vi "Set All Plot Visibility (WFGraph).vi"(8 "error in (no error)":errorcluster, 10 "All Visible?":bool, 11 "WFGraph in":refnum<vi>) -> (0 "error out":errorcluster)   [LabVIEW 2019, in "Instrument.Lockin.lvlib" / "Instrument UI.Lockin.lvclass"]
uses:
  Instrument UI.Lockin.lvclass
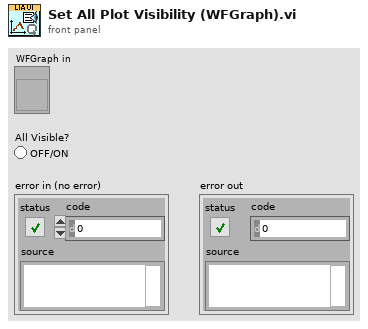
[diagram p1: front panel]
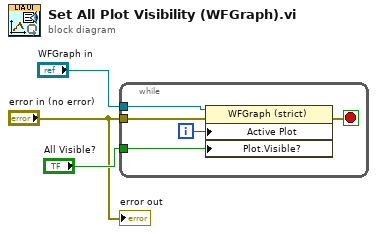
[diagram p0: block diagram]
diagram:
  n1 = while {
    tunnel: "WFGraph in" -> [w5]
    tunnel: "error in (no error)" -> [w6]
    tunnel: "All Visible?" -> [w7]
    i -> [w8]
    stop <- w4 stop-if-true
    n2 = property on="Property Node" class="WFGraph (strict)"(reference=w5, error in=w6, "Active Plot"=w8, "Plot.Visible?"=w7) -> (error out=w4:errorcluster)  [unwired: 1 out]
  }
  "error out" <- "error in (no error)"
